vi "monitoring_center.vi"() -> ()   [LabVIEW 2026]
panel:
  in  "Browse":bool
  out "Array":cluster{i32[], "p":dbl[]}[](array[cluster])
  out "XY Graph":cluster{i32[], "p":dbl[]}[](graph)
  in  "Nodes":T1(array[cluster])
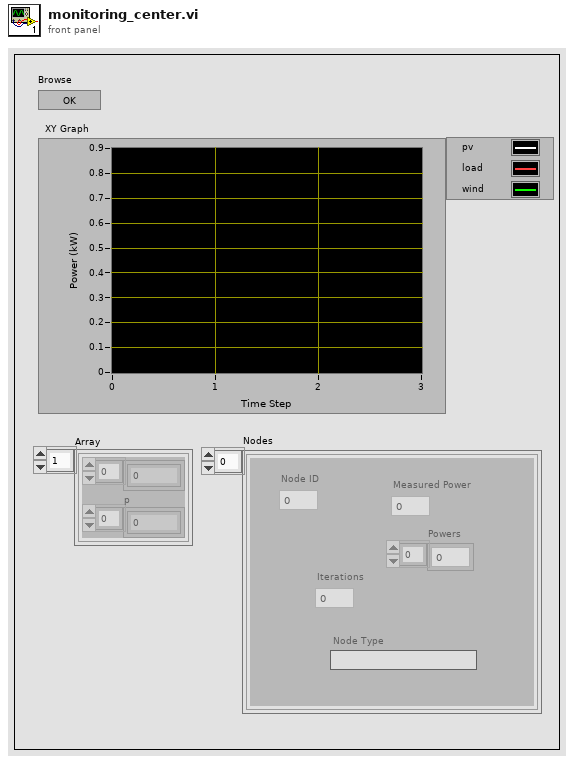
[diagram p1: front panel]
types:
  T1 = cluster{"node_id":i32, "measured_power":dbl, "iterations":i32, "node_type":string, "p":dbl[]}[]
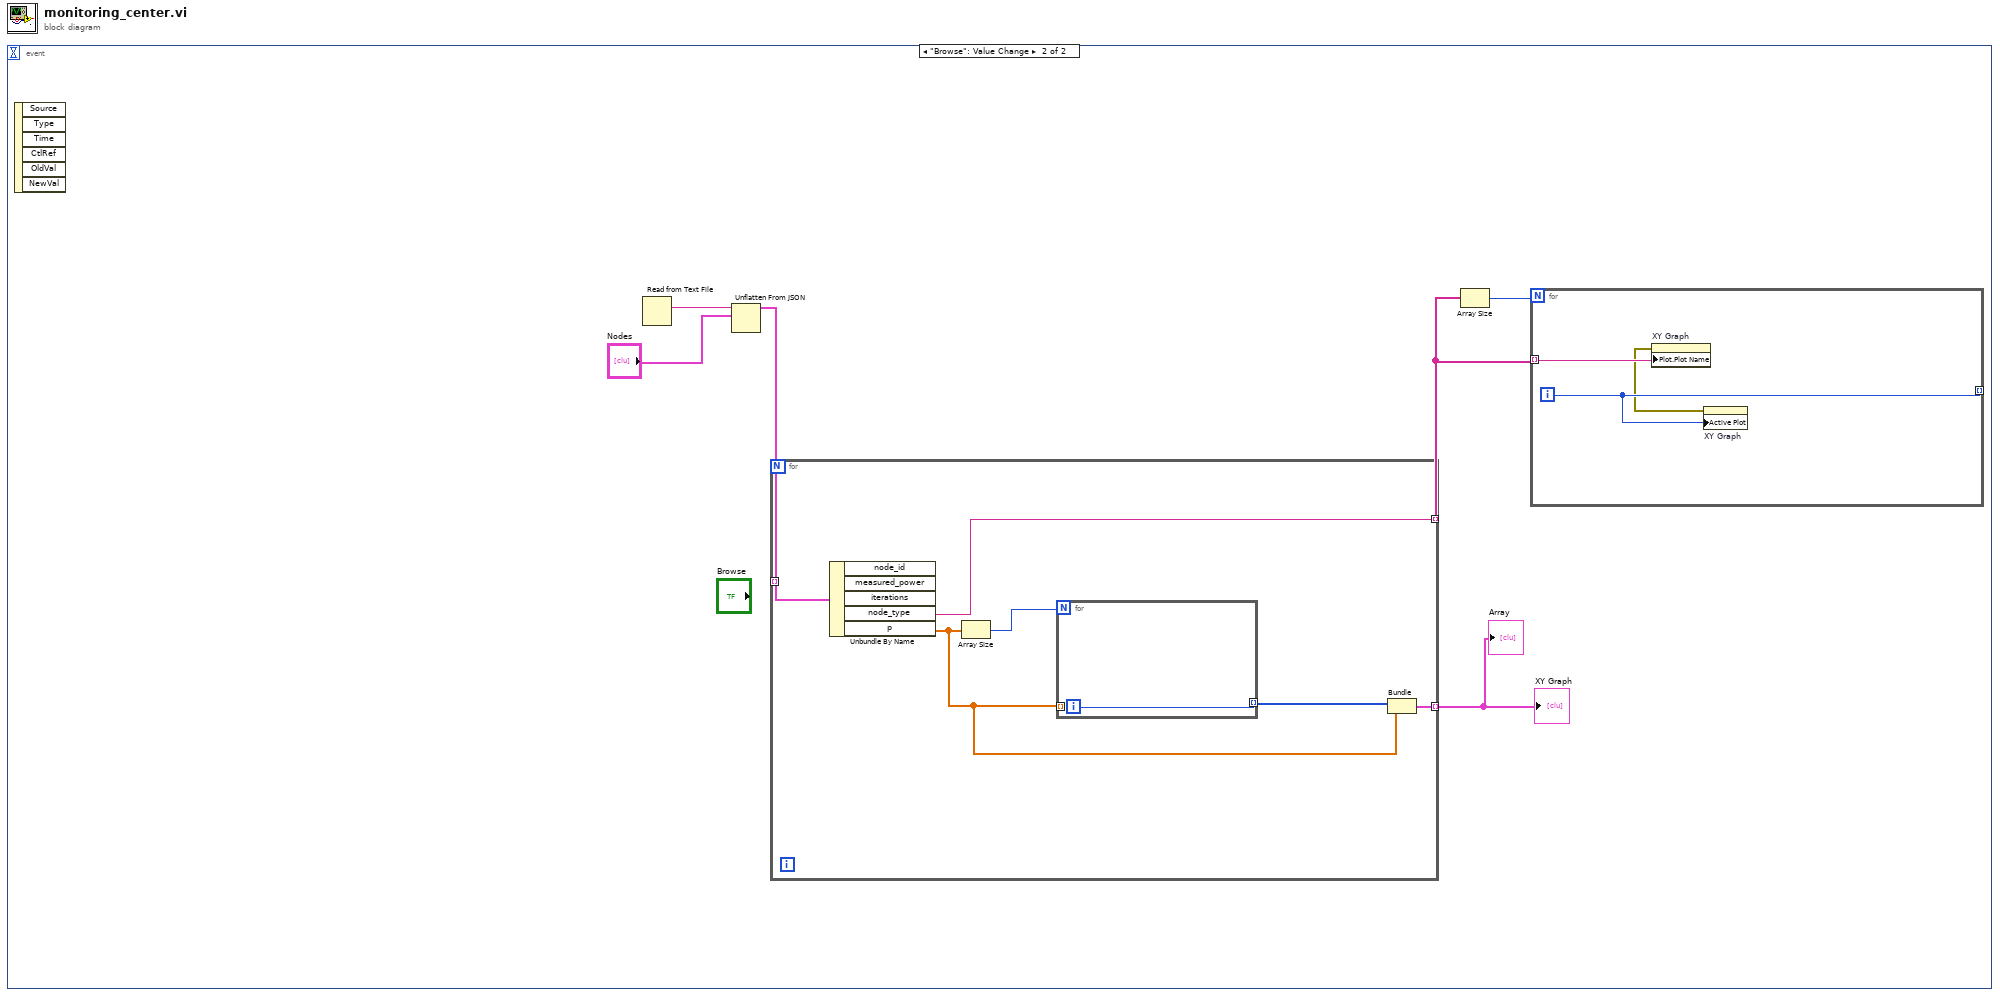
[diagram p0: block diagram]
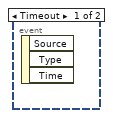
[diagram p2: hidden frame]
diagram:
  n1 = event shown="[1] \"Browse\": Value Change" {
    selector: _ -> [_ _]
    dyn-events: _ -> [_ _]
    timeout: _ -> [_ _]
    event Timeout {
      n2 = event-data() -> ()  [unwired: 1 in, 3 out]
    }
    event "Browse": Value Change {
      n3 = event-data() -> ()  [unwired: 1 in, 6 out]
      n4 = Read from Text File() -> (text=w6:string)  [unwired: 4 in, 3 out]
      n5 = Unflatten From JSON(JSON string=w6, type and defaults="Nodes") -> (value=w4:T1)  [unwired: 5 in, 1 out]
      n6 = for {
        tunnel: w4 -> [w15] mode=indexing
        tunnel: [w12] -> w3 mode=indexing
        tunnel: [w10] -> w1 mode=indexing
        n7 = Unbundle By Name(w15) -> ("node_type"=w10:string, "p"=w11:dbl[])  [unwired: 3 out]
        n8 = Array Size(array=w11) -> (size(s)=w14:i32)
        n9 = for {
          N: w14 -> [_]
          tunnel: w11 -> [_] mode=indexing
          tunnel: [w16] -> w13 mode=indexing
          i -> [w16]
        }
        n10 = Bundle(w13, "p"=w11) -> (w12:cluster{i32[], "p":dbl[]})  [unwired: 1 in]
      }
      "XY Graph" <- w3
      "Array" <- w3
      n11 = Array Size(array=w1) -> (size(s)=w2:i32)
      n12 = for {
        N: w2 -> [_]
        tunnel: [w8] -> _ mode=indexing
        tunnel: w1 -> [w9] mode=indexing
        i -> [w8]
        n13 = property on="XY Graph" class="XYGraph (strict)"("Active Plot"=w8) -> (error out=w7:errorcluster)  [unwired: 2 in, 1 out]
        n14 = property on="XY Graph" class="XYGraph (strict)"(error in=w7, "Plot.Plot Name"=w9) -> ()  [unwired: 1 in, 2 out]
      }
    }
  }
